vi "Clear and Focus Input.vi"(8 "error in":errorcluster, 11 "Input Ref":refnum<vi>) -> (0 "error out":errorcluster)   [LabVIEW 2026]
doc: "Empties a string control and gives it the key focus, so the user can type the next entry straight away. Used by the ATM main VI on User Input whenever it asks for an account number or an amount. The control must be enabled first: a disabled control takes no key focus. Writing Value fires no Value Change event.\n\nError behaviour: if error in carries an error, the control is not changed and the error is passed to error out."
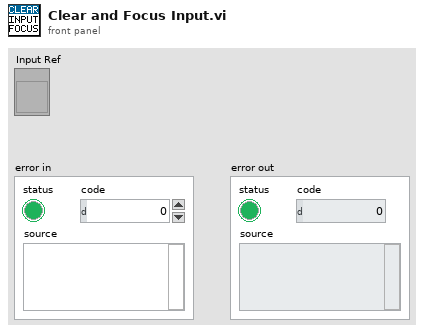
[diagram p1: front panel]
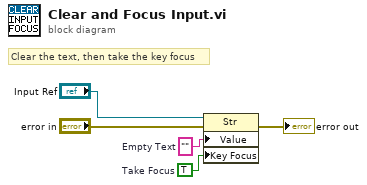
[diagram p0: block diagram]
diagram:
  w2 = TRUE  # Take Focus
  w3 = ""  # Empty Text
  # "Clear the text, then take the key focus"
  n1 = property class="Str"(reference="Input Ref", error in="error in", "Value"=w3, "Key Focus"=w2) -> (error out=→"error out":errorcluster)  [unwired: 1 out]
